vi "Compare Parameters With Refresh Dialog.vi"(8 "error in":errorcluster, 9 "refresh button":bool, 10 "selected parameters file":path caption="path to parameters xml", 11 "configuration files page data in":T1 {"custom device ref" format="%.0x"}) -> (0 "error out":errorcluster, 3 "configuration files page data out":T1 {"custom device ref" format="%.0x"})   [LabVIEW 2020, in "AIM ARINC 429 System Explorer.lvlib" / "Implementation.lvlib"]
uses:
  Implementation.lvlib
  Import/ARINC 429 Import.lvlib
  Scripting/AIM/AIM ARINC 429 Scripting.lvlib
  Types/Browse Button.ctl
  Types/Path Control.ctl
  <vilib>/NI VeriStand/Custom Device API/Custom Device Item Ref.ctl
  <vilib>/NI VeriStand/Custom Device API/Custom Device API.lvlib
  Types/Configuration Files Page Data.ctl
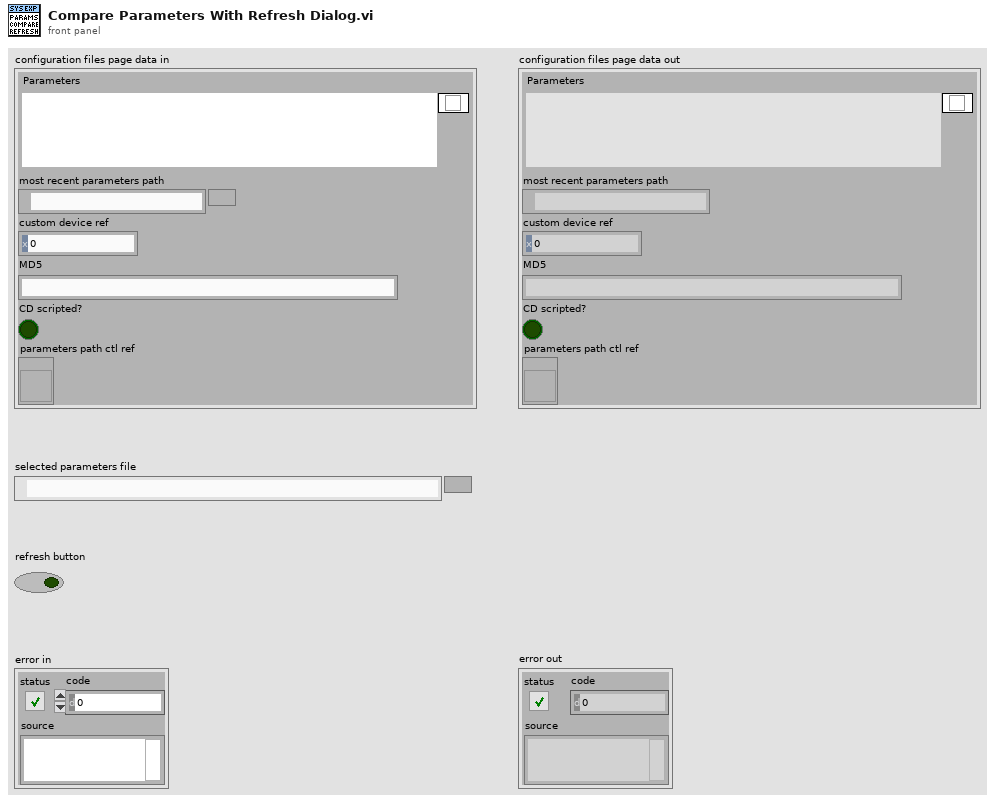
[diagram p1: front panel]
types:
  T1 = typedef "AIM ARINC 429 System Explorer.lvlib/Implementation.lvlib/Configuration Files Page Data.ctl" = cluster{"Parameters":T2, "most recent parameters path":path, "custom device ref":T4, "MD5":string, "CD scripted?":bool, "parameters path ctl ref":refnum<vi>}
  T2 = typedef "AIM ARINC 429 System Explorer.lvlib/Implementation.lvlib/Path Control.ctl" = cluster{"file path":path, "Browse":T3}
  T3 = typedef "AIM ARINC 429 System Explorer.lvlib/Implementation.lvlib/Browse Button.ctl" = bool
  T4 = typedef "Custom Device API.lvlib/Custom Device Item Ref.ctl" = u64
  T5 = typedef "VS Channels Definition for All Labels on Hardware Channel.ctl" = cluster{"hardware channel":i32, "direction":T6, "labels":T7[], "speed":T12}
  T6 = typedef "Direction.ctl" = enum16{"Rx", "Tx"}
  T7 = typedef "VS Channels Definition for Label.ctl" = cluster{"label (Dec)":u32, "parameters":T8[], "SDI value":u8, "SDI enabled":bool, "transfer type":T11, "create timestamp":bool, "transmit period":u32}
  T8 = typedef "VS Channel Definition for Parameter.ctl" = cluster{"name":string, "unit":string, "Parameter":T9}
  T9 = typedef "Parameter Definition.ctl" = cluster{"start index":i32, "size":i32, "encoding":T10, "signed":bool, "scale multiplier":dbl, "scale offset":dbl, "default value":dbl}
  T10 = typedef "Encoding and Decoding.lvlib/Encoding.ctl" = enum16{"BNR", "BCD", "Discrete"}
  T11 = typedef "Transfer Type.ctl" = enum16{"Scheduled", "Acyclic", "Block", "Strobe"}
  T12 = typedef "Transfer Speed.ctl" = enum16{"LO (12.5 kb/s)", "HI (100 kb/s)"}
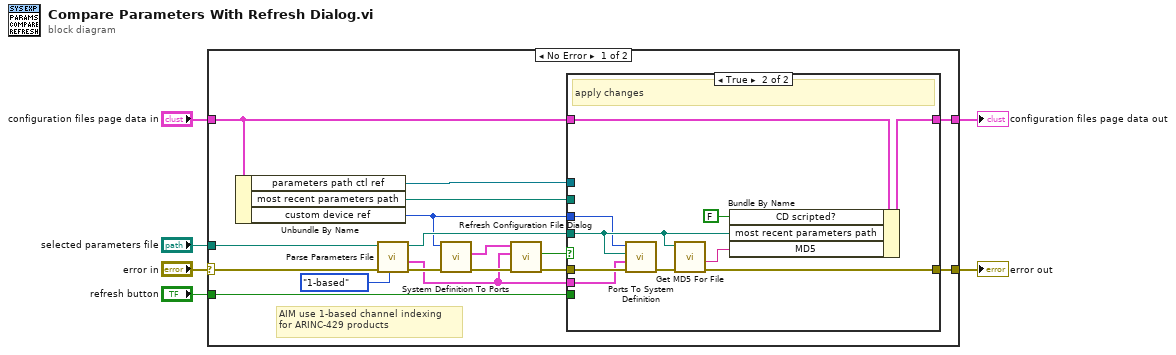
[diagram p0: block diagram]
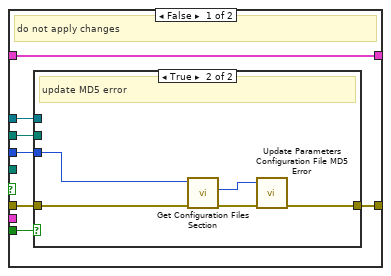
[diagram p2: hidden frame]
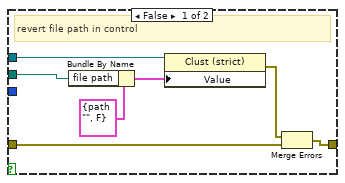
[diagram p3: hidden frame]
diagram:
  n1 = case shown="No Error" "error in" {
    selector: "error in" -> [w23 w54]
    tunnel: [w22 w54] -> w5
    tunnel: "configuration files page data in" -> [w20 w53]
    tunnel: [w19 w53] -> w3
    tunnel: "selected parameters file" -> [w21 _]
    tunnel: "refresh button" -> [w18 _]
    frame No Error {
      # "AIM use 1-based channel indexing\nfor ARINC-429 products"
      n2 = Unbundle By Name(w20) -> ("parameters path ctl ref"=w8:refnum<vi>, "most recent parameters path"=w9:path, "custom device ref"=w10:T4)
      n3 = call "Parse Parameters File.vi"("ch indexing (0-based)"=enum16{"0-based", "1-based"}."1-based", "error in"=w23, "path to XML document"=w21) -> ("error out"=w17:errorcluster, "ports"=w11:T5[], "path to XML document out"=w12:path)  [unwired: 6 in]
      n4 = call "System Definition To Ports.vi"("error in"=w17, "custom device ref"=w10) -> ("error out"=w16:errorcluster, "ports"=w15:T5[])  [unwired: 7 in, 1 out]
      n5 = call "Refresh Configuration File Dialog.vi"("error in"=w16, "new ports"=w11, "current ports"=w15) -> ("error out"=w13:errorcluster, "apply changes"=w14:bool)  [unwired: 7 in]
      n6 = case shown="True" w14 {
        tunnel: w13 -> [w29 w52]
        tunnel: w12 -> [_ w46]
        tunnel: w11 -> [_ w51]
        tunnel: [w30 w47] -> w22
        tunnel: w20 -> [w28 w49]
        tunnel: [w28 w50] -> w19
        tunnel: w18 -> [w27 _]
        tunnel: w10 -> [w26 w44]
        tunnel: w9 -> [w25 _]
        tunnel: w8 -> [w24 _]
        frame False {
          # "do not apply changes"
          n7 = case shown="True" w27 {
            tunnel: [w35 w40] -> w30
            tunnel: w29 -> [w33 w39]
            tunnel: w26 -> [_ w38]
            tunnel: w25 -> [w32 _]
            tunnel: w24 -> [w31 _]
            frame False {
              # "revert file path in control"
              n8 = Bundle By Name(cluster=T2 {"file path"=path "", "Browse"=FALSE} ("Value"), "file path"=w32) -> (w36:T2)
              n9 = property class="Clust (strict)"(reference=w31, "Value"=w36) -> (error out=w34:errorcluster)  [unwired: 1 in, 1 out]
              n10 = Merge Errors(w34, w33) -> (w35:errorcluster)
            }
            frame True {
              # "update MD5 error"
              n11 = call "Get Configuration Files Section.vi"("error in"=w39, "custom device ref"=w38) -> ("error out"=w41:errorcluster, "configuration files ref"=w42:T4)  [unwired: 7 in, 1 out]
              n12 = call "Update Parameters Configuration File MD5 Error.vi"("error in"=w41, "configuration files ref"=w42) -> ("error out"=w40:errorcluster)  [unwired: 8 in, 1 out]
            }
          }
        }
        frame True {
          # "apply changes"
          n13 = call "Ports To System Definition.vi"("error in"=w52, "ports"=w51, "parameter configuration file path"=w46, "custom device ref"=w44) -> ("error out"=w48:errorcluster)  [unwired: 6 in, 1 out]
          n14 = call "Get MD5 For File.vi"("error in"=w48, "path"=w46) -> ("error out"=w47:errorcluster, "MD5"=w45:string)  [unwired: 8 in]
          n15 = Bundle By Name(cluster=w49, "CD scripted?"=FALSE, "most recent parameters path"=w46, "MD5"=w45) -> (w50:T1)
        }
      }
    }
    frame Error {
    }
  }
  "error out" <- w5
  "configuration files page data out" <- w3
